vi "FX_Check.vi"(10 "error in (no error)":errorcluster, 11 "RX":string) -> (2 "error out":errorcluster, 3 "Data":string)   [LabVIEW 2018]
doc: "Use this template to build a VI to use as a subVI."
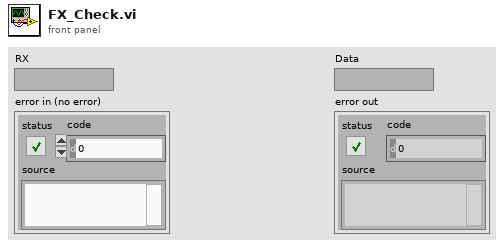
[diagram p1: front panel]
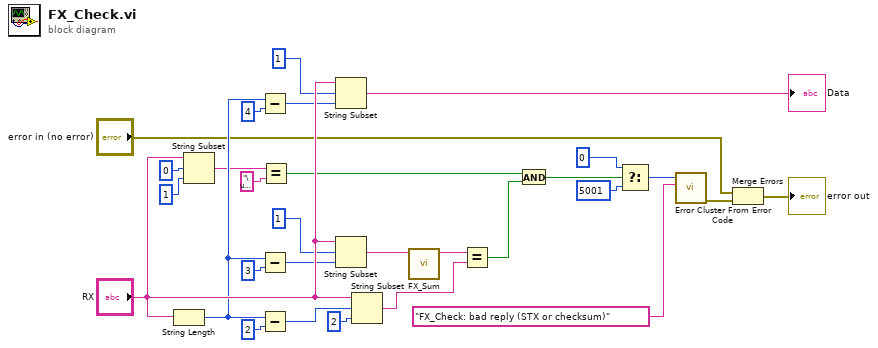
[diagram p0: block diagram]
diagram:
  n1 = String Length(string="RX") -> (length=w26:i32)
  n2 = String Subset(string="RX", offset (0)=0, length (rest)=1 ("length (rest)")) -> (substring=w13:string)
  n3 = Subtract(x=w26, y=4) -> (x-y=w17:i32)
  n4 = Subtract(x=w26, y=3) -> (x-y=w23:i32)
  n5 = Subtract(x=w26, y=2) -> (x-y=w21:i32)
  n6 = Equal?(x=w13, y="\u0002") -> (x = y?=w11:bool)
  n7 = String Subset(string="RX", offset (0)=1, length (rest)=w17) -> (substring=→"Data":string)
  n8 = String Subset(string="RX", offset (0)=1, length (rest)=w23) -> (substring=w16:string)
  n9 = String Subset(string="RX", offset (0)=w21, length (rest)=2 ("length (rest)")) -> (substring=w14:string)
  n10 = call "FX_Sum.vi"("Body"=w16) -> ("SS"=w15:string)  [unwired: 10 in]
  n11 = Equal?(x=w15, y=w14) -> (x = y?=w10:bool)
  n12 = And(x=w11, y=w10) -> (x .and. y?=w9:bool)
  n13 = Select(t=0, s=w9, f=5001) -> (s? t:f=w6:i32)
  n14 = call <vilib>:"Error Cluster From Error Code.vi"("error message (\"\")"="FX_Check: bad reply (STX or checksum)", "error code (0)"=w6) -> ("error out"=w3:errorcluster)  [unwired: 7 in]
  n15 = Merge Errors("error in (no error)", w3) -> (→"error out":errorcluster)
